vi "Documentation.vi"() -> (0 "Author":string, 1 "History":string, 2 "Version":string, 3 "Description":string)   [LabVIEW 2021, in "CAN_Reader_NIXNET_Plugin.lvlib"]
uses:
  CAN_Reader_NIXNET_Plugin.lvlib
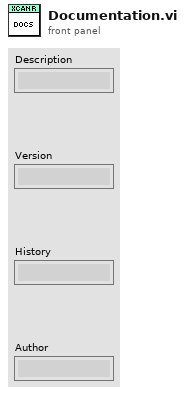
[diagram p1: front panel]
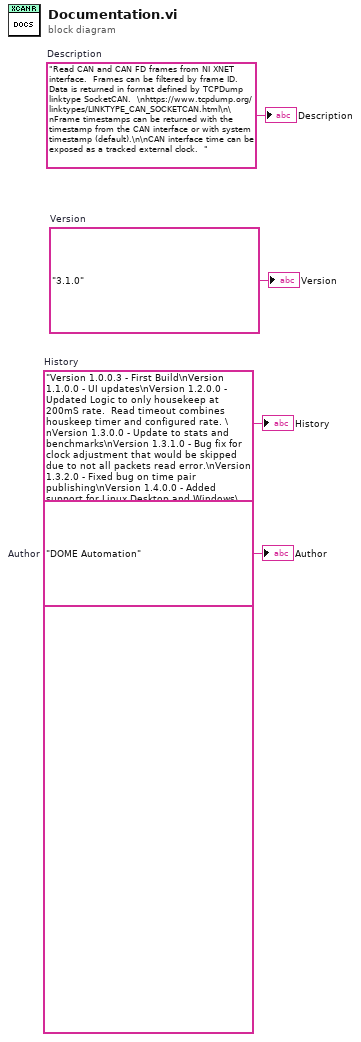
[diagram p0: block diagram]
diagram:
  w1 = "DOME Automation"  # Author
  w2 = "Version 1.0.0.3 - First Build\nVersion 1.1.0.0 - UI updates\nVersion 1.2.0.0 - Updated Logic to only housekeep at 200mS rate.  Read timeout combines houskeep timer and configured rate. \nVersion 1.3.0.0 - Update to stats and benchmarks\nVersion 1.3.1.0 - Bug fix for clock adjustment that would be skipped due to not all packets read error.\nVersion 1.3.2.0 - Fixed bug on time pair publishing\nVersion 1.4.0.0 - Added support for Linux Desktop and Windows\nVersion 1.4.1.0 - Windows fix for Timed Loop priority and mute of 9006 warning.  \nVersion 1.4.2.0 - Windows Log timestamp update to use wall clock time\nVersion 1.4.3.0 - Standard support for mute late cycle warnings on Linux and Windows.  Mute gRCP client timeout in UI.\nVersion 1.4.4.0 - Flexible tag linking support added.\nVersion 2.0.0.0 - Update to gRPC core library.\nVersion 2.0.1.0 - Support for Core UI Class update\nVersion 2.0.2.0 - Register gRPC Descriptors set as config option\nVersion 3.0.0.0 - Support for Core Class to Events\nVersion 3.0.1.0 - Include updated CIPC with bug fix for backpressure and Core update with bug fix to handle error from cleanup.\nVersion 3.0.2.0 - Incorporate core update to close plugin on disconnect of CIF manager\nVersion 3.0.4.0 - Memory optimization\nVersion 3.0.5.0 - Bug in LV UI code to flatten config\nVersion 3.0.6.0 - Pull in fix in core reader code for timeout after filter applied.  \nVersion 3.0.7.0 - Incorporate LV gRPC core library updates to fix memory leaks\rVersion 3.1.0.0 - Added support for CAN Status monitoring and improved error on faults."  # History
  w3 = "3.1.0"  # Version
  w4 = "Read CAN and CAN FD frames from NI XNET interface.  Frames can be filtered by frame ID.  Data is returned in format defined by TCPDump linktype SocketCAN.  \nhttps://www.tcpdump.org/linktypes/LINKTYPE_CAN_SOCKETCAN.html\n\nFrame timestamps can be returned with the timestamp from the CAN interface or with system timestamp (default).\n\nCAN interface time can be exposed as a tracked external clock.  "  # Description
  "Description" <- w4
  "Version" <- w3
  "History" <- w2
  "Author" <- w1
